vi "lvmcp_dfir.vi"() -> ()   [LabVIEW 2026]
panel:
  out "error out":errorcluster
  out "CPP Output":string
  in  "Indentation Level":i32
  in  "VI Variable Name":string
  in  "reference":refnum<vi>
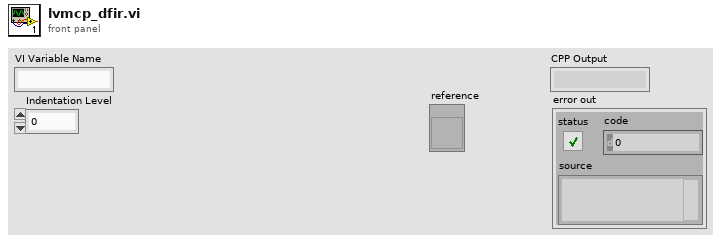
[diagram p1: front panel]
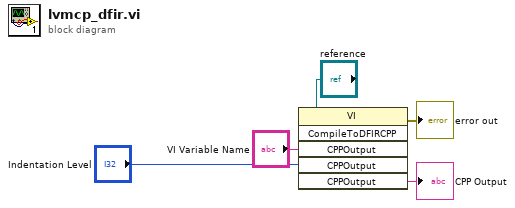
[diagram p0: block diagram]
diagram:
  n1 = invoke class="VI" method="CompileToDFIRCPP"(reference="reference", "CPPOutput"="VI Variable Name", "CPPOutput"="Indentation Level") -> (error out=→"error out":errorcluster, "CPPOutput"=→"CPP Output":string)  [unwired: 3 in, 4 out]
